vi "Actor Core.vi"(8 "error in":errorcluster, 11 "VTU Sim Rig in":refnum<class "VTU Sim Rig.lvclass">) -> (0 "error out":errorcluster, 3 "Actor out":refnum<class "Actor.lvclass">)   [LabVIEW 2026, in "VTU Sim Rig.lvclass"]
doc: "<p>(<strong>Filename</strong>: <span class=\"dnl\">Actor Framework.lvlib:Actor.lvclass:Actor Core.vi</span>)</p>\n<p>Receives messages to the actor, reacts to them, and initiates any error handling that may shut the actor down.</p>\n<p>Descendant classes may override this VI to append parallel tasks for the actor to complete while it handles messages. Overrides use the <a href=\"nihelplauncher://docs/csh?context=lvcore_glang_udclass\">Call Parent Class Method</a> node.</p>"
uses:
  VTU Sim Rig.lvclass
  <vilib>/ActorFramework/Actor/Actor.lvclass
  src/Rig/Rig.lvclass
  VTU Sim Rig.lvclass/VTU Sim Rig.ctl
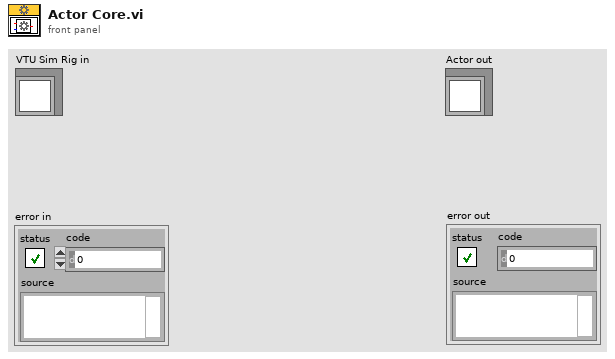
[diagram p1: front panel]
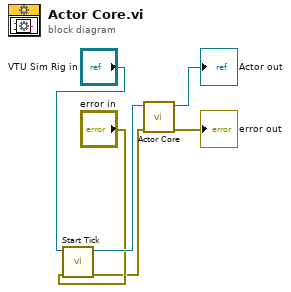
[diagram p0: block diagram]
diagram:
  n1 = call "Start Tick.vi"("error in"="error in", "Actor in"="VTU Sim Rig in") -> ("error out"=w1:errorcluster, "Actor out"=w3:refnum<class "VTU Sim Rig.lvclass">)  [unwired: 8 in]
  n2 = call-parent "Actor Core.vi"("error in"=w1, "Actor in"=w3) -> ("error out"=→"error out":errorcluster, "Actor out"=→"Actor out":refnum<class "Actor.lvclass">)  [unwired: 8 in]
